vi "Element Init.vi"(7 "VolatusAPI":refnum<class "VolatusAPI.lvclass">, 8 "error in (no error)":errorcluster, 10 "JSON":string, 11 "NumericCommandButton in":refnum<class "NumericCommandButton.lvclass">) -> (0 "error out":errorcluster, 3 "NumericCommandButton out":refnum<class "NumericCommandButton.lvclass">)   [LabVIEW 2025, in "VolatusGUIElements.lvlib" / "NumericCommandButton.lvclass"]
uses:
  NumericCommandButton.lvclass
  Volatus/VolatusAPI/VolatusAPI.lvclass
  JSON.ctl
  lv-vecto/Vecto/Group DBL/Group DBL.lvclass
  NumericCommandButton.lvclass/NumericCommandButton.ctl
  7a38387e-77ae-4eb8-b58d-e47934876bff.vi
  <vilib>/JDP Science/JSONtext/JSON text to Variant.vi
  <vilib>/JDP Science/JSONtext/LVClass Serializer/JSONtext LVClass Serializer.lvclass
  C:/dev/volatus/mts-volatus-super/libs/lv-vecto/Vecto/Group/Group.lvclass
  C:/dev/volatus/mts-volatus-super/libs/lv-vecto/Vecto/Group DBL/Group DBL.lvclass
  Volatus/Numeric Command/Numeric Command.lvclass
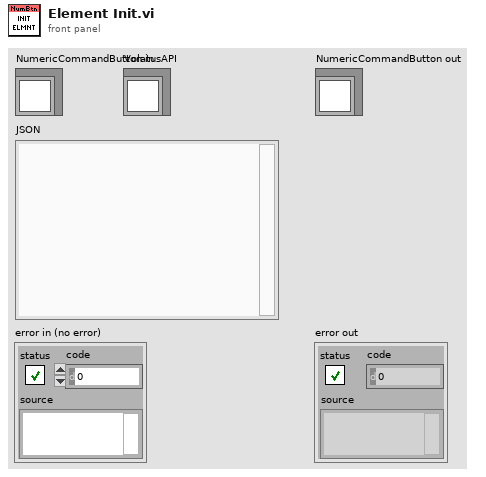
[diagram p1: front panel]
types:
  T1 = typedef "VolatusGUIElements.lvlib/NumericCommandButton.lvclass/JSON.ctl" = cluster{"Channel":string, "Value":dbl}
  T2 = typedef "VectoConfig.lvlib/Channel Info.ctl" = cluster{"Name":string, "Group":string, "Owning Node":string, "Owning Task":string, "Resource":string}
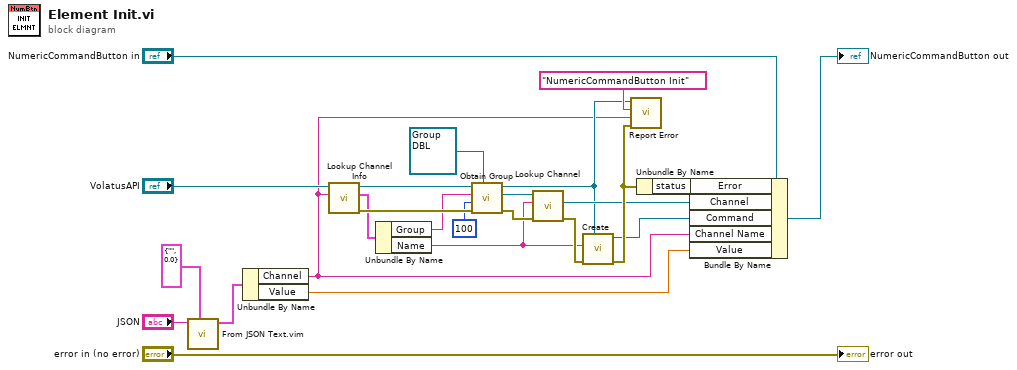
[diagram p0: block diagram]
diagram:
  n1 = call "From JSON Text.vim"("Data Type and Default Value"=T1 {"Channel"="", "Value"=0.0} ("JSON"), "JSON"="JSON") -> ("Data out"=w20:T1)  [unwired: 8 in, 1 out]
  n2 = Unbundle By Name(w20) -> ("Channel"=w1:string, "Value"=w6:dbl)
  n3 = call "Lookup Channel Info.vi"("Channel Name"=w1, "VolatusAPI in"="VolatusAPI") -> ("error out"=w16:errorcluster, "Channel Info"=w13:T2, "VolatusAPI out"=w15:refnum<class "VolatusAPI.lvclass">)  [unwired: 5 in, 2 out]
  n4 = Unbundle By Name(w13) -> ("Group"=w14:string, "Name"=w10:string)
  n5 = call "Obtain Group.vi"("Group Type (Abstract)"=refnum<class "Group DBL.lvclass"> refnum ("Vecto.lvlib:Group.lvclass"), "error in (no error)"=w16, "Timeout ms (5000)"=u32 100, "Group Name"=w14, "VolatusAPI in"=w15) -> ("error out"=w17:errorcluster, "Group"=w18:refnum<class "Group DBL.lvclass">, "VolatusAPI out"=w4:refnum<class "VolatusAPI.lvclass">)  [unwired: 4 in]
  n6 = call "Lookup Channel.vi"("error in (no error)"=w17, "Channel Name"=w10, "Group in"=w18) -> ("error out"=w24:errorcluster, "Channel"=w8:refnum<class "Channel DBL.lvclass">)  [unwired: 6 in, 1 out]
  n7 = call "Create.vi"("VolatusAPI"=w4, "error in (no error)"=w24, "Channel"=w10) -> ("error out"=w25:errorcluster, "Numeric Command out"=w7:refnum<class "Numeric Command.lvclass">)  [unwired: 7 in]
  n8 = call "Report Error.vi"("error in (no error)"=w25, "Message"=w1, "Context"="NumericCommandButton Init", "VolatusAPI in"=w4) -> ()  [unwired: 6 in, 2 out]
  n9 = Unbundle By Name(w25) -> ("status"=w3:bool)
  n10 = Bundle By Name(cluster="NumericCommandButton in", "Error"=w3, "Channel"=w8, "Command"=w7, "Channel Name"=w1, "Value"=w6) -> (→"NumericCommandButton out":refnum<class "NumericCommandButton.lvclass">)
  "error out" <- "error in (no error)"
